vi "SendUDP.vi"(0 "Arg3":u8, 1 "IP":string, 3 "Port":dbl, 5 "Arg4":u8, 7 "Arg5":u8, 9 "Arg6":u8, 11 "Arg7":u8) -> ()   [LabVIEW 2024]
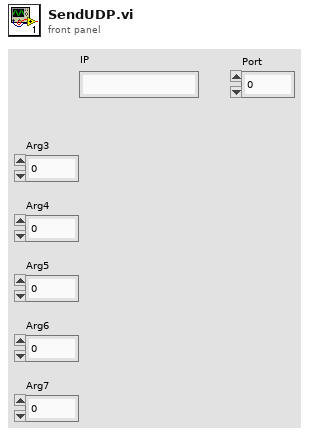
[diagram p1: front panel]
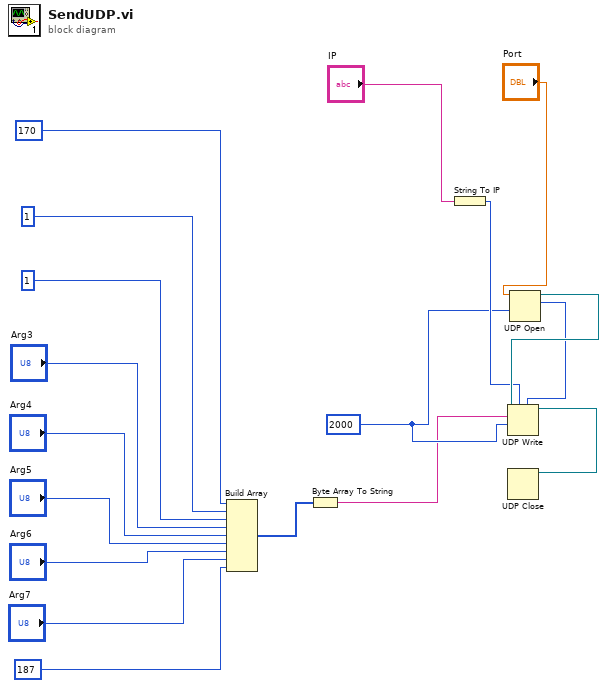
[diagram p0: block diagram]
diagram:
  w15 = 2000 ("timeout ms (25000)")
  n1 = Build Array(u8 170, 1, 1, "Arg3", "Arg4", "Arg5", "Arg6", "Arg7", 187) -> (w12:i32[])
  n2 = Byte Array To String(unsigned byte array=w12) -> (string=w13:string)
  n3 = String To IP(1:"IP") -> (0:w16:u32)
  n4 = UDP Open(9:w15, 11:"Port") -> (port=w18:refnum<k16>, 2:w14:u16)  [unwired: 3 in, 1 out]
  n5 = UDP Write(address=w16, port or service name=w14, connection ID=w18, data in=w13, 9:w15) -> (3:w17:refnum<k16>)  [unwired: 1 in, 1 out]
  n6 = UDP Close(connection ID=w17) -> ()  [unwired: 1 in, 2 out]
